vi "FuncVI-Sqrt.vi"(5 "InstanceRef":T2, 9 "arg list":T1[](array[typedef]) {"num" format="%.2f"}) -> (0 "error out":bool, 3 "result":T1 {"num" format="%.2f"})   [LabVIEW 2021]
doc: "::: CalcExpress Toolkit :::\nCopyright (c) 2000-2026 Konstantin Shifershteyn. All rights reserved."
uses:
  cetypes.llb/CalcExpress Function Argument Info.ctl
  cetypes.llb/CalcExpress Instance RefNum.ctl
panel:
  in  "max arg num":i32=1
  in  "min arg num":i32=1
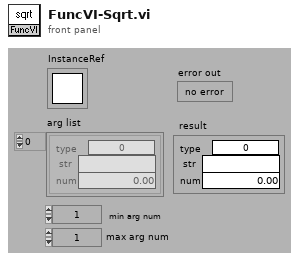
[diagram p1: front panel]
types:
  T1 = typedef "CalcExpress Function Argument Info.ctl" = cluster{"type":u32, "str":string, "num":dbl}
  T2 = typedef "CalcExpress Instance RefNum.ctl" = refnum<k1>
  T3 = enum16{"DBL scalar", "CDB scalar", "DBL array", "CDB array", "ERROR"}
  T4 = typedef "CalcExpress Data Type.ctl" = enum32{"String", "DBL Number", "identifier", "1D Array of DBL", "2D Array of DBL", "CDB Number", "1D Array of CDB", "2D Array of CDB", "1D Array of String", "2D Array of String", "Unknown data type"}
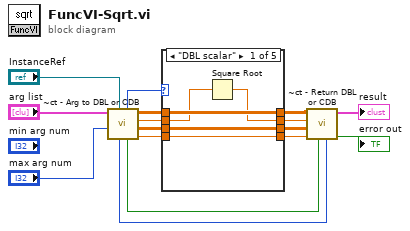
[diagram p0: block diagram]
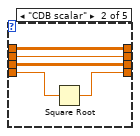
[diagram p2: hidden frame]
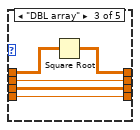
[diagram p3: hidden frame]
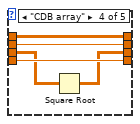
[diagram p4: hidden frame]
diagram:
  n1 = call "~ct - Arg to DBL or CDB.vi"("InstanceRef"="InstanceRef", "max args"="max arg num", "args list"="arg list") -> ("CDB"=w9:cdb, "2D CDB"=w10:cdb[][], "DBL"=w8:dbl, "2D DBL"=w7:dbl[][], "error out"=w12:bool, "category"=w2:T3, "arg type"=w11:T4)  [unwired: 2 in]
  n2 = case shown="\"DBL scalar\"" w2 {
    tunnel: w10 -> [w20 w25 w31 w33 w37]
    tunnel: w9 -> [w19 w23 w30 w34 w38]
    tunnel: w8 -> [w18 w24 w29 w35 w39]
    tunnel: w7 -> [w21 w26 w28 w36 w40]
    tunnel: [w21 w26 w27 w36 w40] -> w6
    tunnel: [w17 w24 w29 w35 w39] -> w5
    tunnel: [w20 w25 w31 w32 w37] -> w4
    tunnel: [w19 w22 w30 w34 w38] -> w3
    frame "DBL scalar" {
      n3 = Square Root(x=w18) -> (sqrt(x)=w17:dbl)
    }
    frame "CDB scalar" {
      n4 = Square Root(x=w23) -> (sqrt(x)=w22:cdb)
    }
    frame "DBL array" {
      n5 = Square Root(x=w28) -> (sqrt(x)=w27:dbl[][])
    }
    frame "CDB array" {
      n6 = Square Root(x=w33) -> (sqrt(x)=w32:cdb[][])
    }
    frame "ERROR" {
    }
  }
  n7 = call "~ct - Return DBL or CDB.vi"("type"=w11, "error in"=w12, "CDB"=w3, "2D CDB"=w4, "DBL"=w5, "2D DBL"=w6) -> ("error out"=→"error out":bool, "result"=→"result":T1)  [unwired: 4 in]
